vi "Get sound from wave file.vi"(6 "init":bool, 7 "cyclic playing":bool=TRUE, 8 "error in":errorcluster, 9 "Sound Rate":enum16{"11025", "22050", "44100"}(ring), 10 "buffer size (samples)":i32=8192, 11 "wave file":path) -> (0 "error out":errorcluster, 1 "EOF":bool, 2 "sound portion":dbl[](array[numeric]), 3 "wave file out":path, 4 "delay (ms)":u32)   [LabVIEW 2021]
doc: "The VI reads sound from a file. The VI returns sounds in sequential blocks of given size to simulate work of a sound divice.\n\n::: CalcExpress Toolkit :::\nCopyright (c) 2000-2026 Konstantin Shifershteyn. All rights reserved."
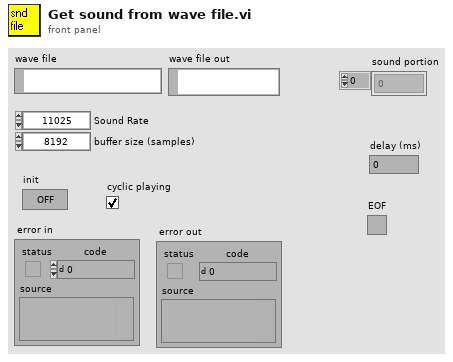
[diagram p1: front panel]
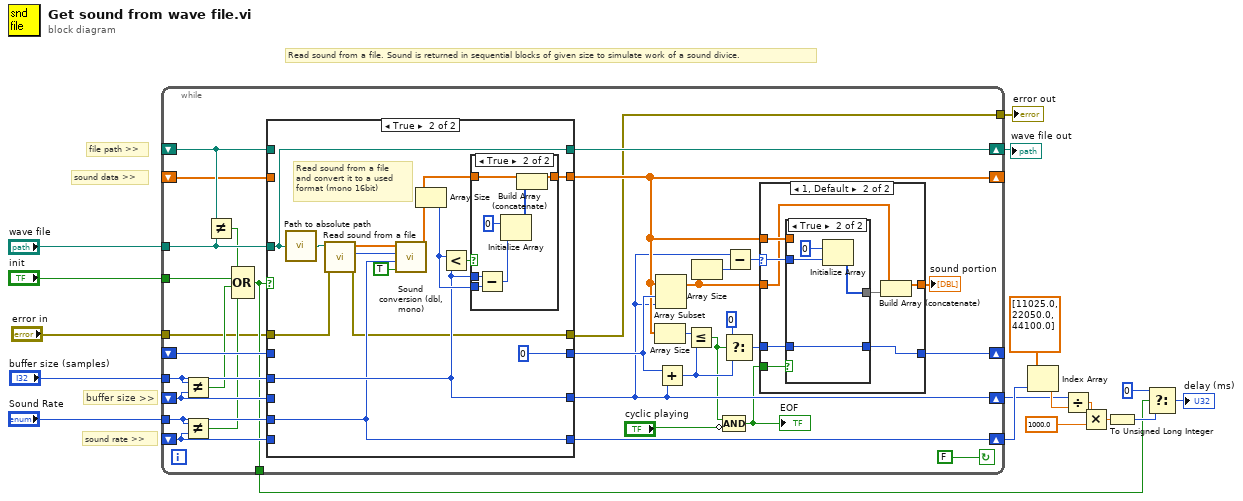
[diagram p0: block diagram]
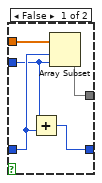
[diagram p3: hidden frame]
diagram:
  # "Read sound from a file. Sound is returned in sequential blocks of given size to simulate work of a sound divice."
  # "file path >>"
  # "sound data >>"
  # "sound rate >>"
  # "buffer size >>"
  n1 = while {
    tunnel: [w22] -> w4
    tunnel: "init" -> [w23]
    shift-left: _ -> [w35]
    shift-right: [w36] -> w9
    tunnel: "buffer size (samples)" -> [w32]
    shift-left: _ -> [w33]
    shift-right: [w38] -> w8
    shift-left: _ -> [w47]
    shift-right: [w42] -> _
    shift-left: _ -> [w48]
    shift-right: [w41] -> _
    tunnel: "Sound Rate" -> [w34]
    tunnel: "wave file" -> [w49]
    shift-left: _ -> [w51]
    shift-right: [w50] -> w10
    tunnel: "error in" -> [w20]
    tunnel: [w19] -> w1
    stop <- FALSE continue-if-true
    n2 = Not Equal?(x=w32, y=w33) -> (x != y?=w31:bool)
    n3 = Not Equal?(x=w34, y=w35) -> (x != y?=w30:bool)
    n4 = Not Equal?(x=w51, y=w49) -> (x != y?=w37:bool)
    n5 = Compound Arithmetic op=OR(w37, w23, w31, w30) -> (w22:bool)
    n6 = case shown="True" w22 {
      tunnel: w51 -> [w76 _]
      tunnel: [w76 w82] -> w50
      tunnel: w49 -> [_ w82]
      tunnel: w34 -> [_ w83]
      tunnel: [w75 w87] -> w41
      tunnel: w48 -> [w75 _]
      tunnel: w20 -> [w74 w78]
      tunnel: [w74 w77] -> w19
      tunnel: w47 -> [w73 _]
      tunnel: [w73 0] -> w46
      tunnel: w33 -> [w72 _]
      tunnel: [w72 w84] -> w38
      tunnel: w32 -> [_ w84]
      tunnel: [w71 w83] -> w36
      tunnel: w35 -> [w71 _]
      frame False {
      }
      frame True {
        # "Read sound from a file\nand convert it to a used\nformat (mono 16bit)"
        n7 = call "Path to absolute path.vi"("path"=w82) -> ("absolute path"=w81:path)  [unwired: 4 in]
        n8 = call "Read sound from a file.vi"("error in"=w78, "path"=w81) -> ("error out"=w77:errorcluster, "rate out"=w79:enum16{"11025", "22050", "44100"}, "Data (mono)"=w80:dbl[])  [unwired: 7 in]
        n9 = call "Sound conversion (dbl, mono).vi"("conver rate? (F)"=TRUE, "output rate"=w83, "file rate"=w79, "sound in"=w80) -> ("sound out"=w86:dbl[])  [unwired: 6 in, 1 out]
        n10 = Array Size(array=w86) -> (size(s)=w88:i32)
        n11 = Less?(x=w88, y=w84) -> (x < y?=w89:bool)
        n12 = case shown="True" w89 {
          tunnel: w84 -> [_ w98]
          tunnel: w88 -> [_ w97]
          tunnel: w86 -> [w91 w95]
          tunnel: [w91 w93] -> w87
          frame False {
          }
          frame True {
            n13 = Subtract(x=w98, y=w97) -> (x-y=w96:i32)
            n14 = Initialize Array(i16 0, w96) -> (w94:i16[])
            n15 = Build Array (concatenate)(w95, w94) -> (w93:dbl[])
          }
        }
      }
    }
    n16 = Array Size(array=w41) -> (size(s)=w45:i32)
    n17 = Array Subset(array=w41, index=w46, length=w38) -> (w44:dbl[])
    n18 = Add(x=w46, y=w38) -> (x+y=w28:i32)
    n19 = Less Or Equal?(x=w45, y=w28) -> (x <= y?=w25:bool)
    n20 = Array Size(array=w44) -> (size(s)=w40:i32)
    n21 = Compound Arithmetic op=AND(w25, invert "cyclic playing") -> (w24:bool)
    "EOF" <- w24
    n22 = Select(t=0 ("f"), s=w25, f=w28) -> (s? t:f=w43:i32)
    n23 = Subtract(x=w38, y=w40) -> (x-y=w39:i32)
    n24 = case shown="1, Default" w39 {
      selector: w39 -> [_ w56]
      tunnel: [w53 w61] -> w29
      tunnel: w44 -> [w53 w54]
      tunnel: w43 -> [w52 w57]
      tunnel: [w52 w58] -> w42
      tunnel: w41 -> [_ w59]
      tunnel: w24 -> [_ w55]
      frame 0 {
      }
      frame 1, Default {
        n25 = case shown="True" w55 {
          tunnel: [w66 w68] -> w60
          tunnel: w59 -> [w65 _]
          tunnel: [w64 w70] -> w58
          tunnel: w57 -> [w63 w70]
          tunnel: w56 -> [w62 w69]
          frame False {
            n26 = Add(x=w62, y=w63) -> (x+y=w64:i32)
            n27 = Array Subset(array=w65, index=w63, length=w62) -> (w66:dbl[])
          }
          frame True {
            n28 = Initialize Array(i16 0, w69) -> (w68:i16[])
          }
        }
        n29 = Build Array (concatenate)(w54, w60) -> (w61:dbl[])
      }
    }
    "sound portion" <- w29
  }
  "wave file out" <- w10
  "error out" <- w1
  n30 = Index Array(array=dbl[] [11025.0, 22050.0, 44100.0], index=w9) -> (element=w12:dbl)
  n31 = Divide(x=w8, y=w12) -> (x/y=w13:dbl)
  n32 = Multiply(x=w13, y=1000.0) -> (x*y=w15:dbl)
  n33 = To Unsigned Long Integer(number=w15) -> (unsigned 32bit integer=w6:u32)
  n34 = Select(t=u32 0, s=w4, f=w6) -> (s? t:f=→"delay (ms)":u32)
